vi "IDS Camera Engine.vi"(0 "IDS Notifier Name":string="Not a Name", 11 "Camera ID":string[](array[string])) -> ()   [LabVIEW 2021]
uses:
  IDS Controls/IDS Parameters.ctl
  IDS Controls/IDS Parameter List.ctl
  IDS Controls/IDS ROI.ctl
  IDS Controls/IDS Actions.ctl
  IDS Controls/IDS Notifier Element.ctl
  <vilib>/vision/Image Controls.llb/IMAQ Image.ctl
  C:/Users/Ries Lab/Documents/Microscope Control from Sheng Account/Microscope-Control/Device Library/Cameras/IDS/IDS LabView Examples/LabVIEW/ueye.NET/uEyeDotNet.dll
  IDS LabView Examples/LabVIEW/ueye.NET/uEyeDotNet.dll
  Camera Controls/Camera IMAQ Key Info.ctl
panel:
  out "Image Key Error":errorcluster
  out "Frame":u32
  in  "Init Camera":bool
  in  "Quit":bool
  in  "Use Display Module":bool
  in  "Capture":bool
  in  "Live Preview":bool
  in  "Get ROI":bool
  in  "Set ROI":bool
  in  "Get Parameter":bool
  in  "Set Parameter":bool
  in  "File Save Path":path
  in  "# of Frames":u32
  in  "ROI Setup":T1
  in  "IDS Parameter":T2
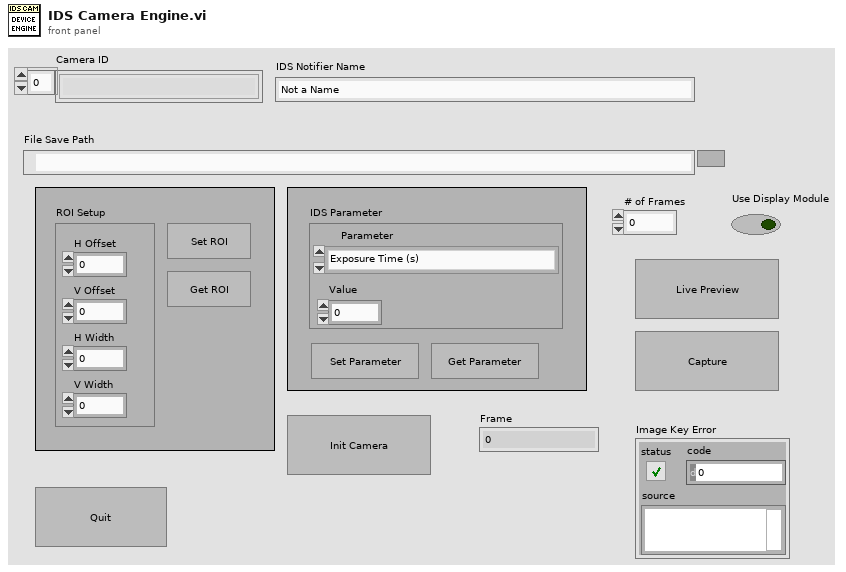
[diagram p1: front panel]
types:
  T1 = typedef "IDS ROI.ctl" = cluster{"H Offset":i32, "V Offset":i32, "H Width":i32, "V Width":i32}
  T2 = typedef "IDS Parameters.ctl" = cluster{"Parameter":T3, "Value":dbl}
  T3 = typedef "IDS Parameter List.ctl" = enum16{"Exposure Time (s)", "Binning", "Gain", "Gamma"}
  T4 = typedef "Image Type" = u32
  T5 = typedef "IDS Notifier Element.ctl" = cluster{"IDS Actions":T6, "Received?":bool, "IDS Parameter":T2, "IDS ROI":T1, "Running?":bool, "File Path":path, "# of frames":u32, "Image Ref":T7, "Error":errorcluster, "Binning":i32}
  T6 = typedef "IDS Actions.ctl" = enum16{"Error Check", "Initialize", "Preview", "Record", "Abort", "Record Settings", "Set Parameter", "Get Parameter", "Set ROI", "Get ROI", "Status", "Quit"}
  T7 = typedef "IMAQ Image.ctl" = refnum<image>
  T8 = typedef "Camera IMAQ Key Info.ctl" = cluster{"Frame":u32, "Sensor Height":i32, "Sensor Width":i32, "ROI Height":i32, "ROI Width":i32, "ROI Enable?":bool, "Bit per Pixel":u8}
  T9 = enum32{"Invalid", "Standard", "Closed", "Hidden", "Minimized", "Maximized"}
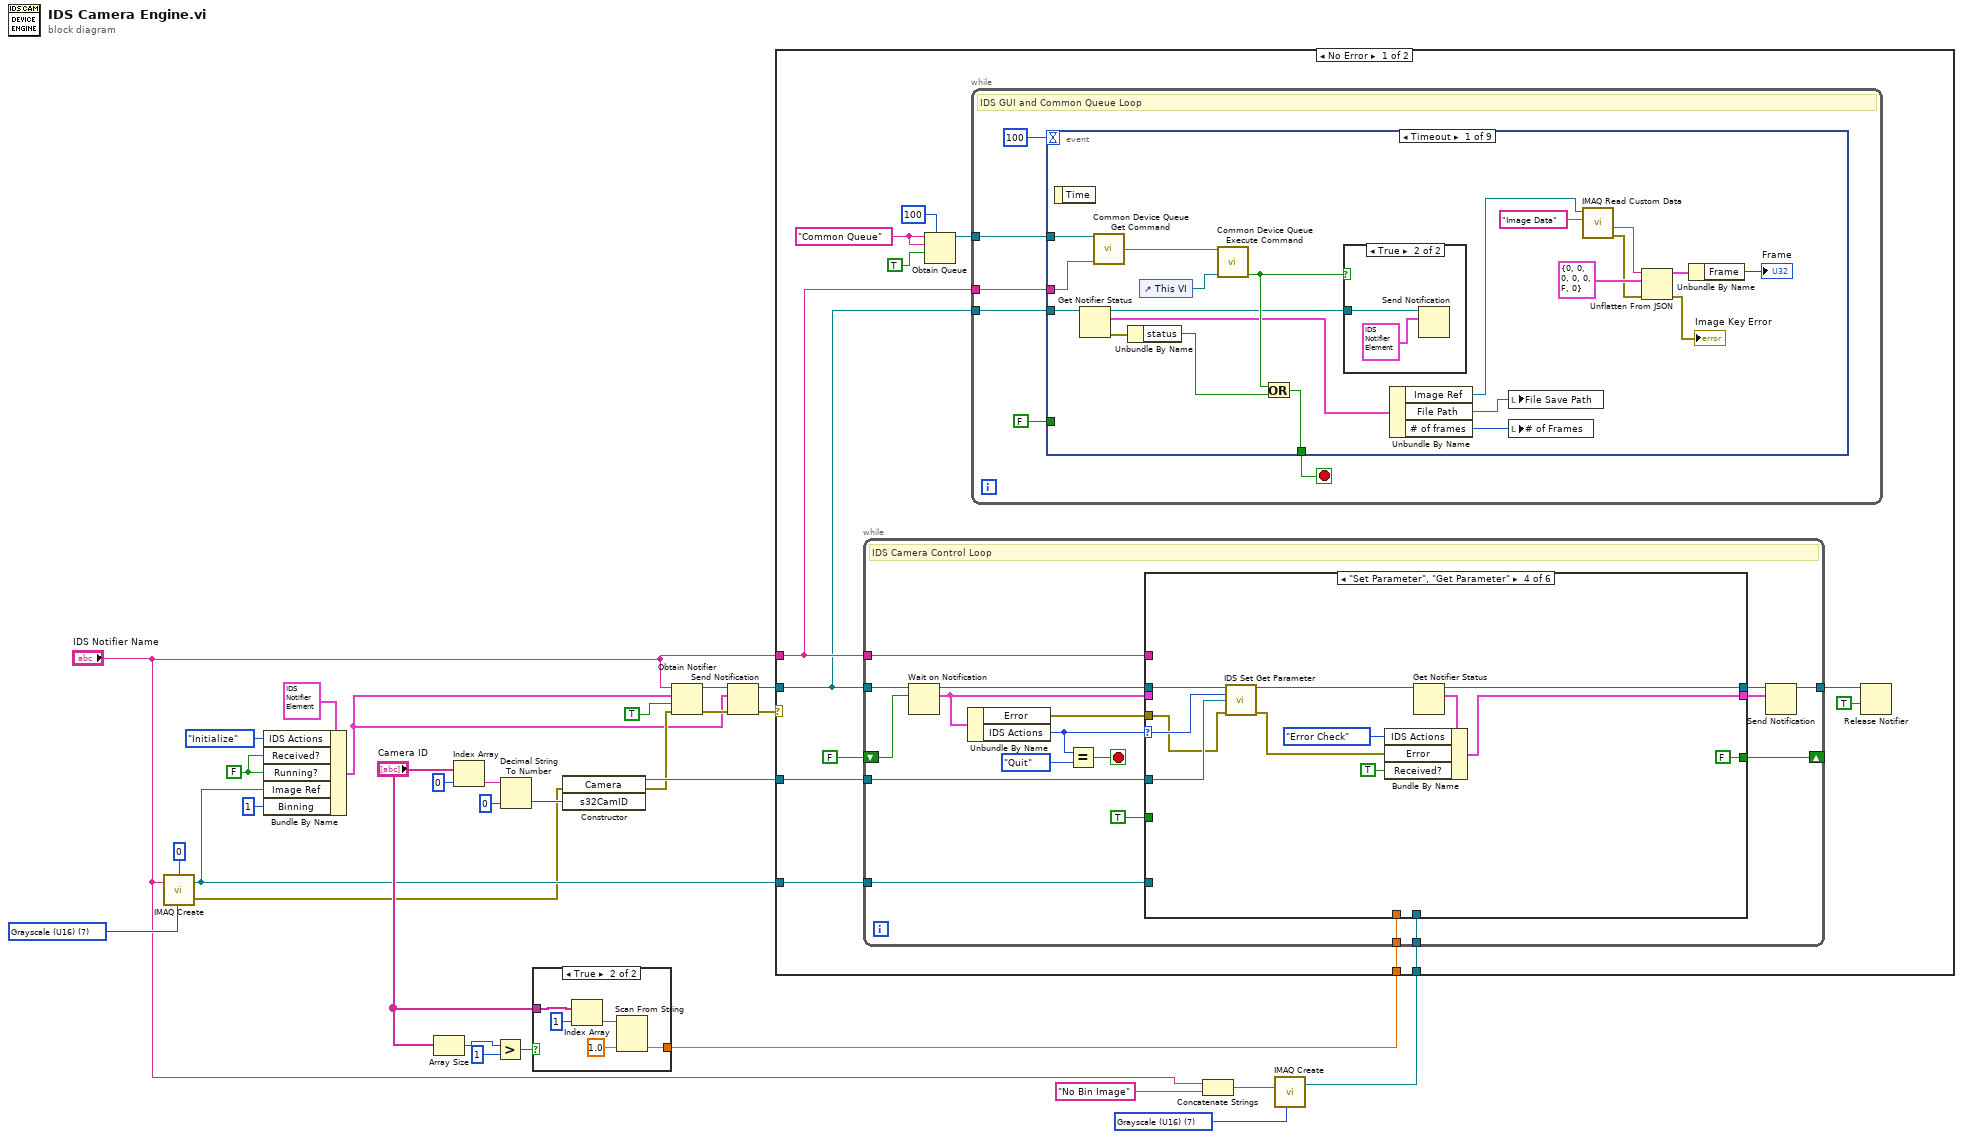
[diagram p0: block diagram]
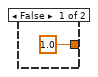
[diagram p2: hidden frame]
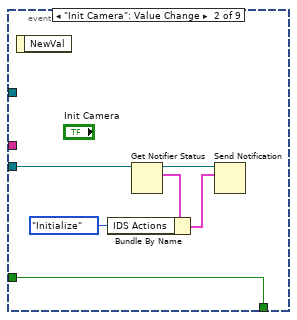
[diagram p4: hidden frame]
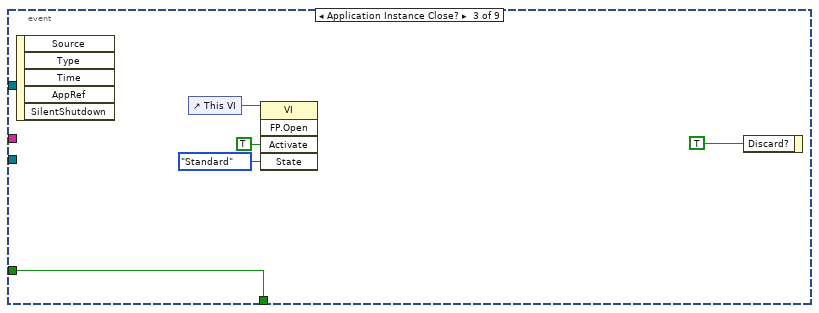
[diagram p5: hidden frame]
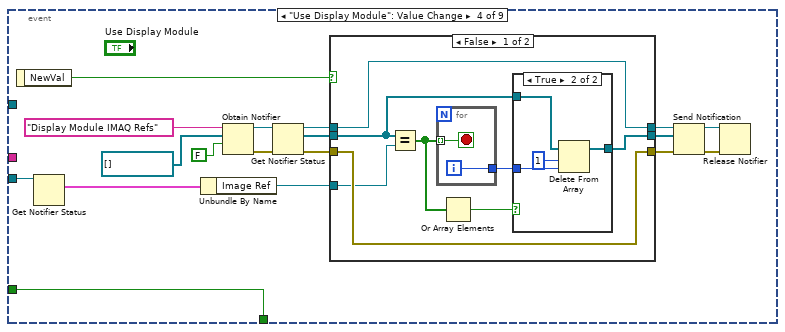
[diagram p6: hidden frame]
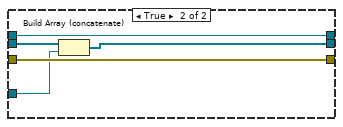
[diagram p8: hidden frame]
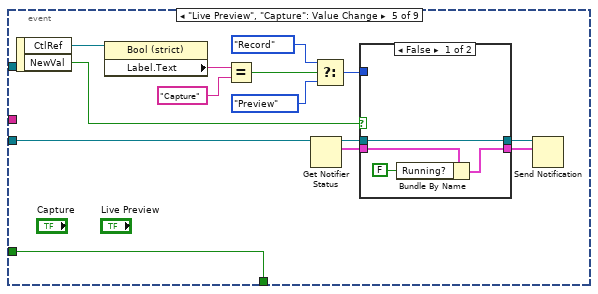
[diagram p9: hidden frame]
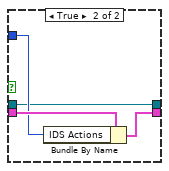
[diagram p10: hidden frame]
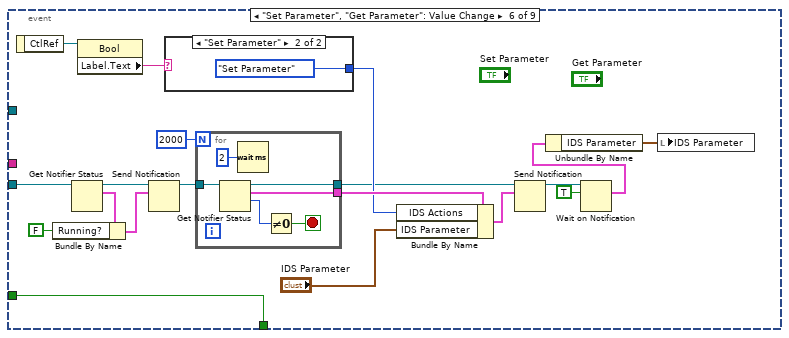
[diagram p11: hidden frame]
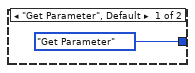
[diagram p12: hidden frame]
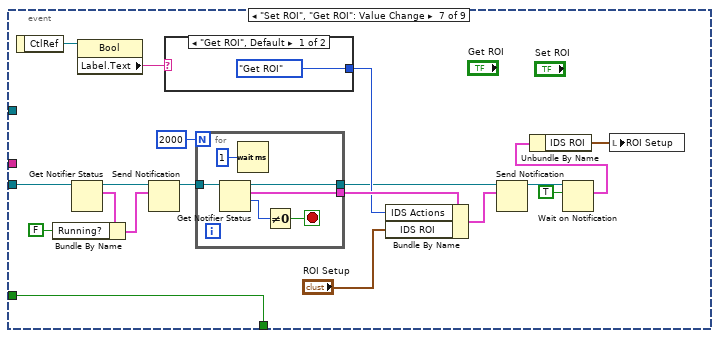
[diagram p13: hidden frame]
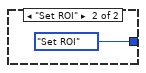
[diagram p14: hidden frame]
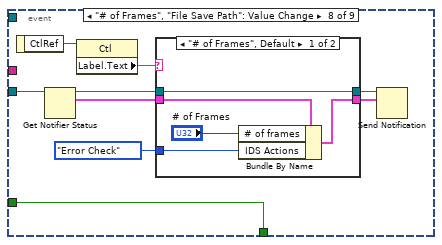
[diagram p15: hidden frame]
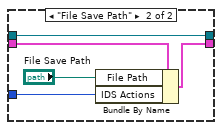
[diagram p16: hidden frame]
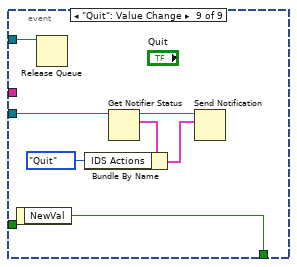
[diagram p17: hidden frame]
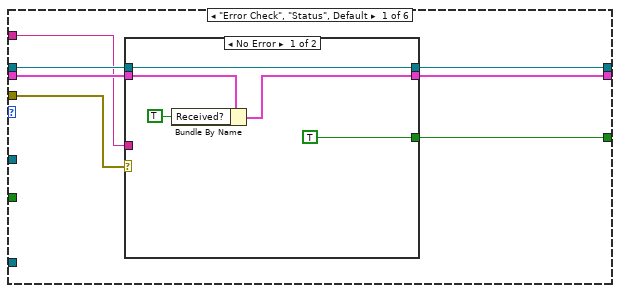
[diagram p18: hidden frame]
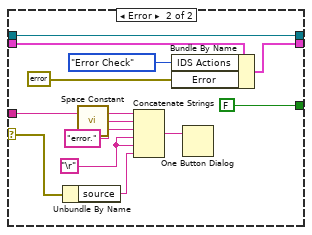
[diagram p19: hidden frame]
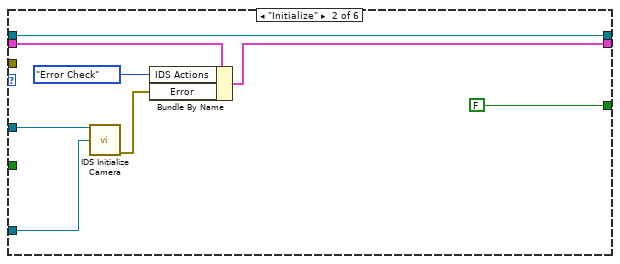
[diagram p20: hidden frame]
diagram:
  w5 = T4 7 items=["Grayscale (U8)", "Grayscale (I16)", "Grayscale (SGL)", "Complex (CSG)", "RGB (U32)", "HSL (U32)", "RGB (U64)", "Grayscale (U16)"] ("Image Type")
  w7 = FALSE ("Received?")
  w20 = T4 7 items=["Grayscale (U8)", "Grayscale (I16)", "Grayscale (SGL)", "Complex (CSG)", "RGB (U32)", "HSL (U32)", "RGB (U64)", "Grayscale (U16)"] ("Image Type")
  n1 = call "IMAQ Create"("Border Size"=0, "Image Name"="IDS Notifier Name", "Image Type"=w20) -> ("New Image"=w19:T7, "error out"=w11:errorcluster)  [unwired: 2 in]
  n2 = Bundle By Name(cluster=T5 {"IDS Actions"=enum."Initialize", "Received?"=FALSE, "IDS Parameter"={"Parameter"=enum."Exposure Time (s)", "Value"=0.0}, "IDS ROI"={"H Offset"=0, "V Offset"=0, "H Width"=0, "V Width"=0}, "Running?"=FALSE, "File Path"=path "", "# of frames"=0, "Image Ref"=refnum, "Error"={"status"=FALSE, "code"=0, "source"=""}, "Binning"=0} ("IDS Camera Cluster"), "IDS Actions"=IDS_Actions."Initialize", "Received?"=w7, "Running?"=w7, "Image Ref"=w19, "Binning"=1) -> (w10:T5)
  n3 = Array Size(array="Camera ID") -> (size(s)=w17:i32)
  n4 = Index Array(array="Camera ID", index=0) -> (element=w23:string)
  n5 = Greater?(x=w17, y=1) -> (0:w16:bool)
  n6 = Decimal String To Number(string=w23, default (0L)=0 ("default (0 I32)")) -> (number=w12:i32)  [unwired: 1 in, 1 out]
  n7 = case shown="True" w16 {
    tunnel: "Camera ID" -> [_ w34]
    tunnel: [1.0 ("default (0 dbl)") w36] -> w18
    frame False {
    }
    frame True {
      n8 = Index Array(array=w34, index=1) -> (element=w35:string)
      n9 = Scan From String(input string=w35, default 1=1.0 ("default (0 dbl)")) -> (output 1=w36:dbl)  [unwired: 3 in, 3 out]
    }
  }
  n10 = constructor class="Camera"(error in=w11, "s32CamID"=w12) -> (reference out=w14:refnum<k24>, error out=w13:errorcluster)  [unwired: 2 in, 2 out]
  n11 = Obtain Notifier(name (unnamed)="IDS Notifier Name", notification data type=w10, create if not found? (T)=TRUE, error in (no error)=w13) -> (notifier out=w29:refnum<notifier>, error out=w28:errorcluster)  [unwired: 1 out]
  n12 = Send Notification(notification=w10, notifier=w29, error in (no error)=w28) -> (notifier out=w27:refnum<notifier>, error out=w26:errorcluster)
  n13 = Concatenate Strings("IDS Notifier Name", "No Bin Image" ("Image Name")) -> (w1:string)
  n14 = call "IMAQ Create"("Image Name"=w1, "Image Type"=w5) -> ("New Image"=w4:T7)  [unwired: 3 in, 1 out]
  n15 = case shown="No Error" w26 {
    selector: w26 -> [_ w351]
    tunnel: w27 -> [w39 w352]
    tunnel: "IDS Notifier Name" -> [w40 w350]
    tunnel: w14 -> [w47 w343]
    tunnel: w19 -> [w46 w342]
    tunnel: w18 -> [w38 _]
    tunnel: w4 -> [w37 _]
    frame No Error {
      w44 = "Common Queue" ("Unique Notifier Name")
      n16 = while {
        tunnel: w39 -> [w245]
        tunnel: [w246] -> w48
        tunnel: w47 -> [w239]
        tunnel: w46 -> [w238]
        shift-right: [w235] -> _
        shift-left: FALSE -> [w237]
        tunnel: w40 -> [w233]
        tunnel: w38 -> [w231]
        tunnel: w37 -> [w230]
        stop <- w247 stop-if-true
        # "IDS Camera Control Loop"
        n17 = Wait on Notification(notifier=w245, ignore previous (F)=w237) -> (notifier out=w244:refnum<notifier>, notification=w243:T5)  [unwired: 2 in, 2 out]
        n18 = Unbundle By Name(w243) -> ("Error"=w232:errorcluster, "IDS Actions"=w242:T6)
        n19 = Equal?(x=w242, y=IDS_Actions."Quit") -> (x = y?=w247:bool)
        n20 = case shown="\"Set Parameter\", \"Get Parameter\"" w242 {
          selector: w242 -> [_ _ w284 w305 w319 _]
          tunnel: w244 -> [w253 w280 w299 w301 w322 w336]
          tunnel: [w252 w280 w296 w310 w313 w336] -> w240
          tunnel: w243 -> [w251 w278 w298 _ _ w334]
          tunnel: w233 -> [w250 _ _ _ _ _]
          tunnel: w239 -> [_ w279 w285 w304 w321 w330]
          tunnel: w238 -> [_ w273 w286 _ w320 w326]
          tunnel: [w249 w275 w295 w306 w312 w332] -> w236
          tunnel: [w254 FALSE FALSE FALSE w323 w335] -> w235
          tunnel: TRUE -> [_ _ _ _ w323 w335]
          tunnel: w232 -> [w248 _ _ w303 _ w327]
          tunnel: w231 -> [_ _ w282 _ _ _]
          tunnel: w230 -> [_ _ w281 _ _ w325]
          frame "Error Check", "Status", Default {
            n21 = case shown="No Error" w248 {
              selector: w248 -> [_ w262]
              tunnel: w251 -> [w257 w272]
              tunnel: [TRUE FALSE] -> w254
              tunnel: [w259 w269] -> w252
              tunnel: w253 -> [w259 w269]
              tunnel: w250 -> [_ w268]
              tunnel: [w255 w264] -> w249
              frame No Error {
                n22 = Bundle By Name(cluster=w257, "Received?"=TRUE) -> (w255:T5)
              }
              frame Error {
                w263 = "\r"
                n23 = Unbundle By Name(w262) -> ("source"=w261:string)
                n24 = call <vilib>:"Space Constant.vi"() -> ("String"=w267:string)
                n25 = Concatenate Strings(w268, w267, "error." ("string"), w263, w263, w261) -> (w265:string)
                n26 = Bundle By Name(cluster=w272, "IDS Actions"=IDS_Actions."Error Check", "Error"=errorcluster {"status"=FALSE, "code"=0, "source"=""}) -> (w264:T5)
                n27 = One Button Dialog(message=w265) -> ()  [unwired: 1 in, 1 out]
              }
            }
          }
          frame "Initialize" {
            n28 = call "IDS Initialize Camera.vi"("Camera ID"=w279, "IDS Cam Img Ref"=w273) -> ("Error Out"=w276:errorcluster)  [unwired: 12 in, 1 out]
            n29 = Bundle By Name(cluster=w278, "IDS Actions"=IDS_Actions."Error Check", "Error"=w276) -> (w275:T5)
          }
          frame "Preview", "Record" {
            w283 = FALSE ("Running?")
            w292 = TRUE ("Received?")
            n30 = Bundle By Name(cluster=w298, "Received?"=w292, "Running?"=w292) -> (w294:T5)
            n31 = Send Notification(notification=w294, notifier=w299) -> (notifier out=w291:refnum<notifier>)  [unwired: 1 in, 1 out]
            n32 = call "IDS Preview Capture.vi"("No Bin Image Ref"=w281, "Pixel Size (µm)"=w282, "Image Ref"=w286, "IDS Camera Ref"=w285, "IDS Actions"=w284, "IDS Notifier"=w291) -> ("Error"=w288:errorcluster, "IDS Notifier"=w290:refnum<notifier>)  [unwired: 4 in]
            n33 = Get Notifier Status(notifier=w290, error in (no error)=w288) -> (notifier out=w296:refnum<notifier>, current notification=w289:T5, error out=w287:errorcluster)  [unwired: 2 out]
            n34 = Bundle By Name(cluster=w289, "IDS Actions"=IDS_Actions."Error Check", "Running?"=w283, "Error"=w287) -> (w295:T5)
            n35 = local write "Capture"(w283) -> ()
          }
          frame "Set Parameter", "Get Parameter" {
            n36 = call "IDS Set Get Parameter.vi"("IDS Notifier"=w301, "IDS Actions"=w305, "IDS Camera Ref"=w304, "Error"=w303) -> ("IDS Notifier"=w311:refnum<notifier>, "Error"=w307:errorcluster)  [unwired: 10 in]
            n37 = Get Notifier Status(notifier=w311) -> (notifier out=w310:refnum<notifier>, current notification=w309:T5)  [unwired: 1 in, 3 out]
            n38 = Bundle By Name(cluster=w309, "IDS Actions"=IDS_Actions."Error Check", "Error"=w307, "Received?"=TRUE) -> (w306:T5)
          }
          frame "Set ROI", "Get ROI" {
            n39 = call "IDS Set Get ROI.vi"("IDS Notifier Ref"=w322, "IDS Actions"=w319, "IDS Camera Ref"=w321, "IDS Image Ref"=w320) -> ("IDS Notifier Ref (Dup)"=w314:refnum<notifier>, "Error"=w315:errorcluster)  [unwired: 10 in]
            n40 = Get Notifier Status(notifier=w314) -> (notifier out=w313:refnum<notifier>, current notification=w318:T5)  [unwired: 1 in, 3 out]
            n41 = Bundle By Name(cluster=w318, "IDS Actions"=IDS_Actions."Error Check", "Error"=w315, "Received?"=TRUE) -> (w312:T5)
          }
          frame "Quit" {
            n42 = invoke class="Camera" method="Exit"(reference=w330, error in=w327) -> (reference out=w331:refnum<k24>, error out=w329:errorcluster)  [unwired: 1 in, 1 out]
            n43 = Close Reference(reference=w331, error in (no error)=w329) -> (error out=w328:errorcluster)
            n44 = Bundle By Name(cluster=w334, "Received?"=TRUE, "Error"=w328) -> (w332:T5)
            n45 = Build Array(w326, w325) -> (w324:T7[])
            n46 = for {
              tunnel: w324 -> [w337] mode=indexing
              n47 = call "IMAQ Dispose"("Image"=w337) -> ()  [unwired: 5 in, 1 out]
            }
          }
        }
        n48 = Send Notification(notification=w236, notifier=w240) -> (notifier out=w246:refnum<notifier>)  [unwired: 1 in, 1 out]
      }
      n49 = Obtain Queue(max queue size (-1, unlimited)=100, name (unnamed)=w44, element data type=w44, create if not found? (T)=TRUE) -> (queue out=w41:refnum<queue>)  [unwired: 1 in, 2 out]
      n50 = while {
        tunnel: w41 -> [w54]
        tunnel: w40 -> [w52]
        tunnel: w39 -> [w53]
        stop <- w51 stop-if-true
        # "IDS GUI and Common Queue Loop"
        n51 = event shown="[0] Timeout" {
          selector: _ -> [_ _ _ _ _ _ _ _ _]
          dyn-events: _ -> [_ _ _ _ _ _ _ _ _]
          timeout: 100 -> [_ _ _ _ _ _ _ _ _]
          tunnel: w54 -> [w70 _ _ _ _ _ _ _ w229]
          tunnel: w53 -> [w69 w83 _ w107 w132 w166 w193 w210 w228]
          tunnel: w52 -> [w68 _ _ _ _ _ _ _ _]
          tunnel: [w67 w84 w89 w90 w141 w168 w195 w212 w223] -> w51
          tunnel: FALSE -> [_ w84 w89 w90 w141 w168 w195 w212 _]
          event Timeout {
            n52 = event-data() -> ()  [unwired: 1 in, 1 out]
            n53 = Get Notifier Status(notifier=w69) -> (notifier out=w71:refnum<notifier>, current notification=w64:T5, error out=w76:errorcluster)  [unwired: 1 in, 2 out]
            n54 = call "Common Device Queue Get Command.vi"("Common Queue"=w70, "Notifier Name"=w68) -> ("Command"=w75:string)  [unwired: 12 in, 1 out]
            n55 = Unbundle By Name(w76) -> ("status"=w73:bool)
            n56 = control-ref of="This VI"() -> (w74:refnum<vi>)
            n57 = call "Common Device Queue Execute Command.vi"("Common Command"=w75, "VI Refnum"=w74) -> ("Quit?"=w72:bool)  [unwired: 12 in, 1 out]
            n58 = Or(x=w72, y=w73) -> (x .or. y?=w67:bool)
            n59 = case shown="True" w72 {
              tunnel: w71 -> [_ w78]
              frame False {
              }
              frame True {
                n60 = Send Notification(notification=T5 {"IDS Actions"=enum."Quit", "Received?"=FALSE, "IDS Parameter"={"Parameter"=enum."Exposure Time (s)", "Value"=0.0}, "IDS ROI"={"H Offset"=0, "V Offset"=0, "H Width"=0, "V Width"=0}, "Running?"=FALSE, "File Path"=path "", "# of frames"=0, "Image Ref"=refnum, "Error"={"status"=FALSE, "code"=0, "source"=""}, "Binning"=0} ("IDS Camera Cluster"), notifier=w78) -> ()  [unwired: 1 in, 2 out]
              }
            }
            n61 = Unbundle By Name(w64) -> ("Image Ref"=w62:T7, "File Path"=w66:path, "# of frames"=w65:u32)
            n62 = local write "File Save Path"(w66) -> ()
            n63 = local write "# of Frames"(w65) -> ()
            n64 = call "IMAQ Read Custom Data"("Key"="Image Data", "Image"=w62) -> ("error out"=w57:errorcluster, "Custom Data Out"=w60:string)  [unwired: 7 in, 1 out]
            n65 = Unflatten From JSON(JSON string=w60, type and defaults=T8 {"Frame"=0, "Sensor Height"=0, "Sensor Width"=0, "ROI Height"=0, "ROI Width"=0, "ROI Enable?"=FALSE, "Bit per Pixel"=0} ("Camera IMAQ Key Info"), error in (no error)=w57) -> (value=w59:T8, error out=→"Image Key Error":errorcluster)  [unwired: 4 in]
            n66 = Unbundle By Name(w59) -> ("Frame"=→"Frame":u32)
          }
          event "Init Camera": Value Change {
            n67 = event-data() -> ()  [unwired: 1 in, 1 out]
            n68 = Get Notifier Status(notifier=w83) -> (notifier out=w79:refnum<notifier>, current notification=w82:T5)  [unwired: 1 in, 3 out]
            n69 = Bundle By Name(cluster=w82, "IDS Actions"=IDS_Actions."Initialize") -> (w80:T5)
            n70 = Send Notification(notification=w80, notifier=w79) -> ()  [unwired: 1 in, 2 out]
          }
          event Application Instance Close? {
            n71 = event-data() -> ()  [unwired: 1 in, 5 out]
            n72 = control-ref of="This VI"() -> (w86:refnum<vi>)
            n73 = invoke class="VI" method="FP.Open"(reference=w86, "Activate"=TRUE ("Activate?"), "State"=T9."Standard") -> ()  [unwired: 2 in, 5 out]
            n74 = event-data("Discard?"=TRUE) -> ()  [unwired: 1 in, 1 out]
          }
          event "Use Display Module": Value Change {
            n75 = event-data() -> ("NewVal"=w92:bool)  [unwired: 1 in]
            n76 = Get Notifier Status(notifier=w107) -> (current notification=w106:T5)  [unwired: 1 in, 4 out]
            n77 = Unbundle By Name(w106) -> ("Image Ref"=w91:T7)
            n78 = Obtain Notifier(name (unnamed)="Display Module IMAQ Refs", notification data type=T7[] [], create if not found? (T)=FALSE) -> (notifier out=w99:refnum<notifier>, error out=w98:errorcluster)  [unwired: 1 in, 1 out]
            n79 = Get Notifier Status(notifier=w99, error in (no error)=w98) -> (notifier out=w100:refnum<notifier>, current notification=w102:T7[], error out=w101:errorcluster)  [unwired: 2 out]
            n80 = case shown="False" w92 {
              tunnel: w100 -> [w115 w125]
              tunnel: w101 -> [w109 w124]
              tunnel: w102 -> [w111 w127]
              tunnel: [w110 w126] -> w105
              tunnel: [w115 w125] -> w103
              tunnel: [w109 w124] -> w104
              tunnel: w91 -> [w108 w123]
              frame False {
                n81 = Equal?(x=w111, y=w108) -> (x = y?=w114:bool[])
                n82 = for {
                  tunnel: w114 -> [w122] mode=indexing
                  tunnel: [w121] -> w112
                  i -> [w121]
                  stop <- w122 stop-if-true
                }
                n83 = Or Array Elements(Boolean array=w114) -> (logical OR=w113:bool)
                n84 = case shown="True" w113 {
                  tunnel: w112 -> [_ w119]
                  tunnel: w111 -> [w116 w118]
                  tunnel: [w116 w117] -> w110
                  frame False {
                  }
                  frame True {
                    n85 = Delete From Array(array=w118, length=1, index=w119) -> (array with subset deleted=w117:T7[])  [unwired: 1 out]
                  }
                }
              }
              frame True {
                n86 = Build Array (concatenate)(w127, w123) -> (w126:T7[])
              }
            }
            n87 = Send Notification(notification=w105, notifier=w103, error in (no error)=w104) -> (notifier out=w97:refnum<notifier>, error out=w96:errorcluster)
            n88 = Release Notifier(notifier=w97, error in (no error)=w96) -> ()  [unwired: 1 in, 3 out]
          }
          event "Live Preview", "Capture": Value Change {
            n89 = event-data() -> ("CtlRef"=w140:refnum<vi>, "NewVal"=w134:bool)  [unwired: 1 in]
            n90 = property class="Bool (strict)"(reference=w140) -> ("Label.Text"=w139:string)  [unwired: 1 in, 2 out]
            n91 = Equal?(x=w139, y="Capture") -> (x = y?=w137:bool)
            n92 = Get Notifier Status(notifier=w132) -> (notifier out=w131:refnum<notifier>, current notification=w130:T5)  [unwired: 1 in, 3 out]
            n93 = Select(t=IDS_Actions."Record" ("y"), s=w137, f=IDS_Actions."Preview" ("y")) -> (s? t:f=w133:T6)
            n94 = case shown="False" w134 {
              tunnel: w133 -> [_ w148]
              tunnel: w131 -> [w143 w147]
              tunnel: w130 -> [w145 w149]
              tunnel: [w143 w147] -> w129
              tunnel: [w142 w146] -> w128
              frame False {
                n95 = Bundle By Name(cluster=w145, "Running?"=FALSE) -> (w142:T5)
              }
              frame True {
                n96 = Bundle By Name(cluster=w149, "IDS Actions"=w148) -> (w146:T5)
              }
            }
            n97 = Send Notification(notification=w128, notifier=w129) -> ()  [unwired: 1 in, 2 out]
          }
          event "Set Parameter", "Get Parameter": Value Change {
            n98 = event-data() -> ("CtlRef"=w167:refnum<vi>)  [unwired: 1 in]
            n99 = Get Notifier Status(notifier=w166) -> (notifier out=w161:refnum<notifier>, current notification=w164:T5)  [unwired: 1 in, 3 out]
            n100 = Bundle By Name(cluster=w164, "Running?"=FALSE) -> (w160:T5)
            n101 = property class="Bool"(reference=w167) -> ("Label.Text"=w165:string)  [unwired: 1 in, 2 out]
            n102 = Send Notification(notification=w160, notifier=w161) -> (notifier out=w159:refnum<notifier>)  [unwired: 1 in, 1 out]
            n103 = case shown="\"Set Parameter\"" w165 {
              tunnel: [IDS_Actions."Get Parameter" ("IDS Actions") IDS_Actions."Set Parameter" ("IDS Actions")] -> w156
              frame "Get Parameter", Default {
              }
              frame "Set Parameter" {
              }
            }
            n104 = for {
              N: 2000 -> [_]
              tunnel: w159 -> [w173]
              tunnel: [w172] -> w155
              tunnel: [w171] -> w158
              stop <- w169 stop-if-true
              n105 = Get Notifier Status(notifier=w173) -> (notifier out=w172:refnum<notifier>, current notification=w171:T5, # waiting=w170:i32)  [unwired: 1 in, 2 out]
              n106 = Wait (ms)(milliseconds to wait=u32 2) -> ()  [unwired: 1 out]
              n107 = Not Equal To 0?(x=w170) -> (x != 0?=w169:bool)
            }
            n108 = Bundle By Name(cluster=w158, "IDS Actions"=w156, "IDS Parameter"="IDS Parameter") -> (w154:T5)
            n109 = Send Notification(notification=w154, notifier=w155) -> (notifier out=w153:refnum<notifier>)  [unwired: 1 in, 1 out]
            n110 = Wait on Notification(notifier=w153, ignore previous (F)=TRUE) -> (notification=w151:T5)  [unwired: 2 in, 3 out]
            n111 = Unbundle By Name(w151) -> ("IDS Parameter"=w150:T2)
            n112 = local write "IDS Parameter"(w150) -> ()
          }
          event "Set ROI", "Get ROI": Value Change {
            n113 = event-data() -> ("CtlRef"=w194:refnum<vi>)  [unwired: 1 in]
            n114 = Get Notifier Status(notifier=w193) -> (notifier out=w188:refnum<notifier>, current notification=w191:T5)  [unwired: 1 in, 3 out]
            n115 = Bundle By Name(cluster=w191, "Running?"=FALSE) -> (w187:T5)
            n116 = property class="Bool"(reference=w194) -> ("Label.Text"=w192:string)  [unwired: 1 in, 2 out]
            n117 = Send Notification(notification=w187, notifier=w188) -> (notifier out=w186:refnum<notifier>)  [unwired: 1 in, 1 out]
            n118 = case shown="\"Get ROI\", Default" w192 {
              tunnel: [IDS_Actions."Get ROI" ("IDS Actions") IDS_Actions."Set ROI" ("IDS Actions")] -> w184
              frame "Get ROI", Default {
              }
              frame "Set ROI" {
              }
            }
            n119 = for {
              N: 2000 -> [_]
              tunnel: w186 -> [w200]
              tunnel: [w199] -> w183
              tunnel: [w198] -> w185
              stop <- w196 stop-if-true
              n120 = Get Notifier Status(notifier=w200) -> (notifier out=w199:refnum<notifier>, current notification=w198:T5, # waiting=w197:i32)  [unwired: 1 in, 2 out]
              n121 = Wait (ms)(milliseconds to wait=u32 1) -> ()  [unwired: 1 out]
              n122 = Not Equal To 0?(x=w197) -> (x != 0?=w196:bool)
            }
            n123 = Bundle By Name(cluster=w185, "IDS Actions"=w184, "IDS ROI"="ROI Setup") -> (w182:T5)
            n124 = Send Notification(notification=w182, notifier=w183) -> (notifier out=w181:refnum<notifier>)  [unwired: 1 in, 1 out]
            n125 = Wait on Notification(notifier=w181, ignore previous (F)=TRUE) -> (notification=w179:T5)  [unwired: 2 in, 3 out]
            n126 = Unbundle By Name(w179) -> ("IDS ROI"=w178:T1)
            n127 = local write "ROI Setup"(w178) -> ()
          }
          event "# of Frames", "File Save Path": Value Change {
            n128 = event-data() -> ("CtlRef"=w211:refnum<vi>)  [unwired: 1 in]
            n129 = Get Notifier Status(notifier=w210) -> (notifier out=w208:refnum<notifier>, current notification=w207:T5)  [unwired: 1 in, 3 out]
            n130 = property class="Ctl"(reference=w211) -> ("Label.Text"=w209:string)  [unwired: 1 in, 2 out]
            n131 = case shown="\"# of Frames\", Default" w209 {
              tunnel: w208 -> [w215 w222]
              tunnel: w207 -> [w217 w221]
              tunnel: [w215 w222] -> w206
              tunnel: [w214 w220] -> w205
              tunnel: IDS_Actions."Error Check" ("IDS Actions") -> [w213 w218]
              frame "# of Frames", Default {
                n132 = Bundle By Name(cluster=w217, "# of frames"="# of Frames", "IDS Actions"=w213) -> (w214:T5)
              }
              frame "File Save Path" {
                n133 = Bundle By Name(cluster=w221, "File Path"="File Save Path", "IDS Actions"=w218) -> (w220:T5)
              }
            }
            n134 = Send Notification(notification=w205, notifier=w206) -> ()  [unwired: 1 in, 2 out]
          }
          event "Quit": Value Change {
            n135 = event-data() -> ("NewVal"=w223:bool)  [unwired: 1 in]
            n136 = Release Queue(queue=w229) -> ()  [unwired: 2 in, 3 out]
            n137 = Get Notifier Status(notifier=w228) -> (notifier out=w227:refnum<notifier>, current notification=w226:T5)  [unwired: 1 in, 3 out]
            n138 = Bundle By Name(cluster=w226, "IDS Actions"=IDS_Actions."Quit") -> (w224:T5)
            n139 = Send Notification(notification=w224, notifier=w227) -> ()  [unwired: 1 in, 2 out]
          }
        }
      }
      n140 = Release Notifier(notifier=w48, force destroy? (F)=TRUE) -> ()  [unwired: 1 in, 3 out]
    }
    frame Error {
      n141 = Release Notifier(notifier=w352, force destroy? (F)=TRUE, error in (no error)=w351) -> (error out=w341:errorcluster)  [unwired: 2 out]
      n142 = invoke class="Camera" method="Exit"(reference=w343, error in=w341) -> (reference out=w344:refnum<k24>, error out=w340:errorcluster)  [unwired: 1 in, 1 out]
      n143 = Close Reference(reference=w344, error in (no error)=w340) -> (error out=w339:errorcluster)
      n144 = call "IMAQ Dispose"("Image"=w342, "error in (no error)"=w339) -> ("error out"=w338:errorcluster)  [unwired: 4 in]
      n145 = Unbundle By Name(w338) -> ("source"=w345:string)
      n146 = call <vilib>:"Space Constant.vi"() -> ("String"=w348:string)
      n147 = Concatenate Strings(w350, w348, "Device Error." ("string"), "\r", w345) -> (w349:string)
      n148 = One Button Dialog(message=w349) -> ()  [unwired: 1 in, 1 out]
    }
  }
